vi "wsCallService.vi"(8 "error in (no error)":errorcluster, 10 "Call Service Data":T1, 11 "References":T2) -> (0 "error out":errorcluster, 3 "Success?":bool)   [LabVIEW 2018, in "HASS-LV-WS_integration.lvlib"]
uses:
  HASS-LV-WS_integration.lvlib
  TypeDef/ReferencesTypeDef.ctl
  TypeDef/QueueTypeDef.ctl
  TypeDef/EventTypeDef.ctl
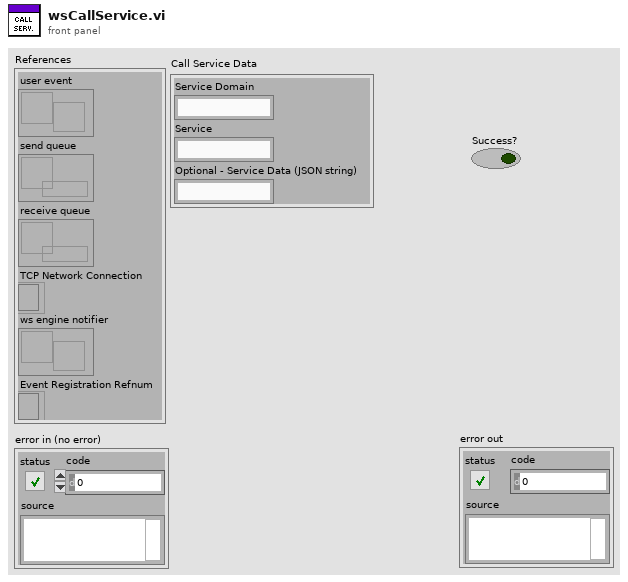
[diagram p1: front panel]
types:
  T1 = cluster{"Service Domain":string, "Service":string, "Optional - Service Data (JSON string)":string}
  T2 = typedef "HASS-LV-WS_integration.lvlib/ReferencesTypeDef.ctl" = cluster{"user event":refnum<user-event>, "send queue":refnum<queue>, "receive queue":refnum<queue>, "TCP Network Connection":refnum<k5>, "ws engine notifier ":refnum<notifier>, "Event Registration Refnum":refnum<event-registration>}
  T3 = typedef "HASS-LV-WS_integration.lvlib/EventTypeDef.ctl" = cluster{"Data":variant, "Command":string}
  T4 = cluster{"id":i32, "type":string, "domain":string, "service":string, "service_data":string}
  T5 = cluster{"id":i32, "type":string, "domain":string, "service":string}
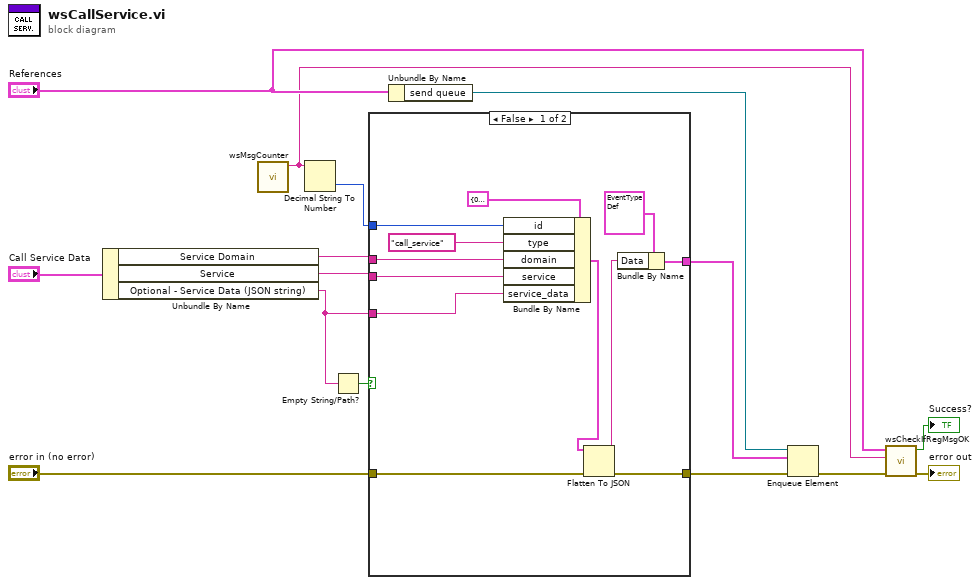
[diagram p0: block diagram]
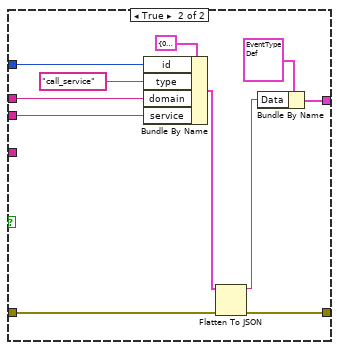
[diagram p2: hidden frame]
diagram:
  n1 = Unbundle By Name("Call Service Data") -> ("Service Domain"=w5:string, "Service"=w4:string, "Optional - Service Data (JSON string)"=w3:string)
  n2 = call "wsMsgCounter.vi"() -> ("msgCounter"=w13:string)  [unwired: 11 in]
  n3 = Decimal String To Number(string=w13) -> (number=w12:i32)  [unwired: 2 in, 1 out]
  n4 = Empty String/Path?(string/path=w3) -> (empty?=w11:bool)
  n5 = case shown="False" w11 {
    tunnel: w12 -> [w26 w37]
    tunnel: w5 -> [w24 w36]
    tunnel: w4 -> [w23 w35]
    tunnel: w3 -> [w22 _]
    tunnel: [w20 w32] -> w10
    tunnel: "error in (no error)" -> [w18 w28]
    tunnel: [w19 w29] -> w1
    frame False {
      n6 = Bundle By Name(cluster=T4 {"id"=0, "type"="", "domain"="", "service"="", "service_data"=""}, "id"=w26, "type"="call_service", "domain"=w24, "service"=w23, "service_data"=w22) -> (w17:T4)
      n7 = Flatten To JSON(anything=w17, error in (no error)=w18) -> (JSON string=w16:string, 11:w19:errorcluster)  [unwired: 1 in]
      n8 = Bundle By Name(cluster=T3 {"Data"=variant, "Command"="Send"} ("element"), "Data"=w16) -> (w20:T3)
    }
    frame True {
      n9 = Bundle By Name(cluster=T5 {"id"=0, "type"="", "domain"="", "service"=""}, "id"=w37, "type"="call_service", "domain"=w36, "service"=w35) -> (w31:T5)
      n10 = Flatten To JSON(anything=w31, error in (no error)=w28) -> (JSON string=w30:string, 11:w29:errorcluster)  [unwired: 1 in]
      n11 = Bundle By Name(cluster=T3 {"Data"=variant, "Command"="Send"} ("element"), "Data"=w30) -> (w32:T3)
    }
  }
  n12 = Unbundle By Name("References") -> ("send queue"=w15:refnum<queue>)
  n13 = Enqueue Element(queue=w15, element=w10, error in (no error)=w1) -> (error out=w9:errorcluster)  [unwired: 1 in, 2 out]
  n14 = call "wsCheckIfRegMsgOK.vi"("error in (no error)"=w9, "msgCounter"=w13, "References"="References") -> ("error out"=→"error out":errorcluster, "Success?"=→"Success?":bool)  [unwired: 6 in, 1 out]
